vi "[ce] Check CE Help Keyword.vi"(11 "keyword for help":string) -> (0 "found":bool, 1 "DIS tag":string, 3 "dup keyword for help":string)   [LabVIEW 2021]
doc: "::: CalcExpress Toolkit :::\nCopyright (c) 2000-2026 Konstantin Shifershteyn. All rights reserved."
uses:
  [ce] CE component paths - Kind of Path Enum.ctl
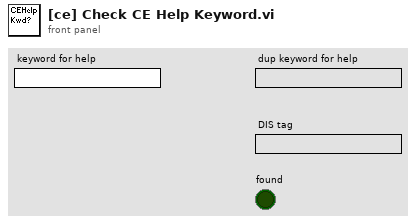
[diagram p1: front panel]
types:
  T1 = typedef "[ce] CE component paths - Kind of Path Enum.ctl" = enum16{"VIs", "FuncVIs", "Help", "Examples", "Project", "Templates"}
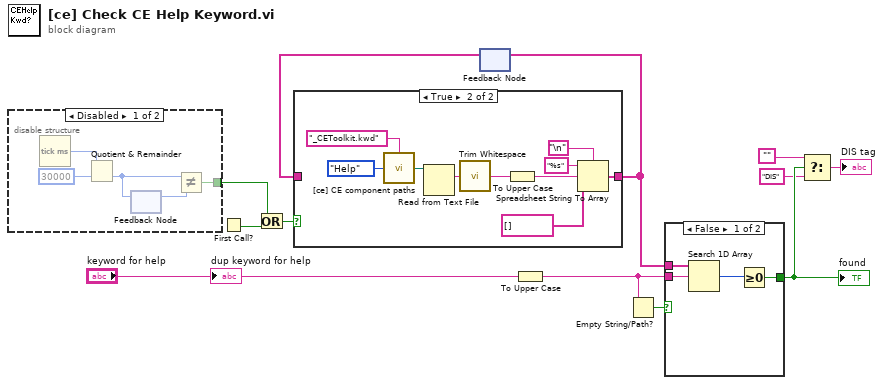
[diagram p0: block diagram]
diagram:
  n1 = disable-structure shown="Disabled" {
    disable-tunnel: [w13 _] -> w8
    frame Disabled {
      n2 = Tick Count (ms)() -> (millisecond timer value=w17:u32)
      n3 = Quotient & Remainder(x=w17, y=u32 30000) -> (floor(x/y)=w15:u32)  [unwired: 1 out]
      n4 = feedback #1() -> (w14:u32)  [unwired: 1 in]
      n5 = feedback-in #1(w15) -> ()
      n6 = Not Equal?(x=w15, y=w14) -> (x != y?=w13:bool)
    }
    frame Enabled {
    }
  }
  n7 = First Call?() -> (First Call?: T/F=w7:bool)
  n8 = Or(x=w8, y=w7) -> (x .or. y?=w12:bool)
  n9 = feedback #2() -> (w10:string[])  [unwired: 1 in]
  n10 = case shown="True" w12 {
    tunnel: [w18 w22] -> w11
    tunnel: w10 -> [w18 _]
    frame False {
    }
    frame True {
      n11 = call "[ce] CE component paths.vi"("kind of path"=[ce]_CE_component_paths_-_Kind_of_Path_Enum."Help", "append path"="_CEToolkit.kwd") -> ("path out"=w26:path)
      n12 = Read from Text File(file (use dialog)=w26) -> (text=w25:string)  [unwired: 3 in, 3 out]
      n13 = call <vilib>:"Trim Whitespace.vi"("string"=w25) -> ("trimmed string"=w20:string)  [unwired: 1 in]
      n14 = To Upper Case(1:w20) -> (0:w19:string)
      n15 = Spreadsheet String To Array(delimiter (Tab)="\n", format string="%s", spreadsheet string=w19, array type (2D Dbl)=string[] []) -> (array=w22:string[])
    }
  }
  n16 = feedback-in #2(w11) -> ()
  n17 = To Upper Case(1:"keyword for help") -> (0:w6:string)
  n18 = Empty String/Path?(string/path=w6) -> (empty?=w9:bool)
  n19 = case shown="False" w9 {
    tunnel: [w31 _] -> w5
    tunnel: w6 -> [w30 _]
    tunnel: w11 -> [w29 _]
    frame False {
      n20 = Search 1D Array(1D array=w29, element=w30) -> (index of element=w32:i32)  [unwired: 1 in]
      n21 = Greater Or Equal To 0?(x=w32) -> (x >= 0?=w31:bool)
    }
    frame True {
    }
  }
  "found" <- w5
  n22 = Select(t="", s=w5, f="DIS") -> (s? t:f=→"DIS tag":string)
  "dup keyword for help" <- "keyword for help"
